vi "Check if Error Occurred.vi"(8 "error in (no error)":errorcluster, 11 "Response header":string) -> (0 "error out":errorcluster, 2 "500 Error":bool, 3 "Error Occurred":bool)   [LabVIEW 2015, in "NI_AWS_Core.lvlib" / "HTTP Request.lvclass"]
doc: "Check the response header to see if there was an error.\nIf an error is found, the AWS_S3_Get_Call_Result.vi may get the details from the response body."
uses:
  HTTP Request.lvclass
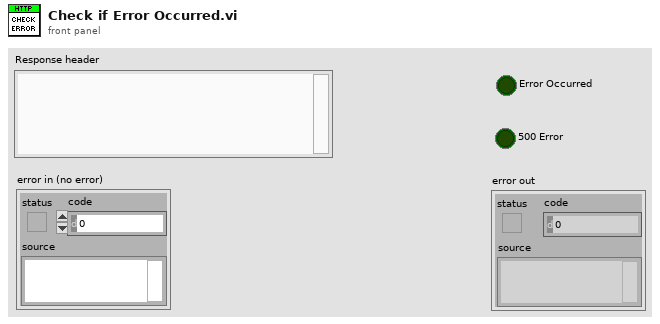
[diagram p1: front panel]
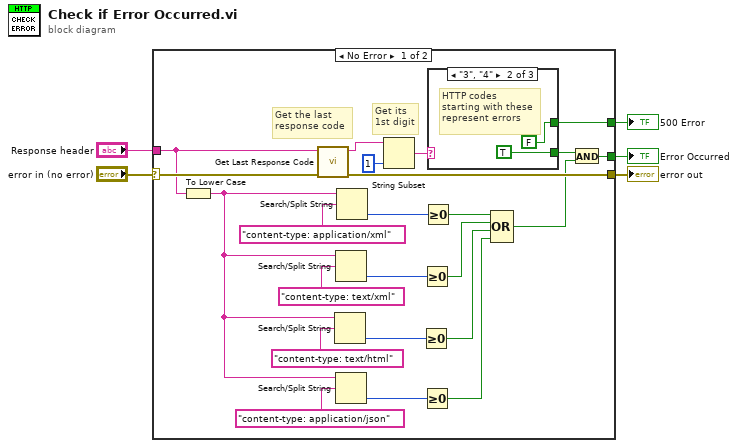
[diagram p0: block diagram]
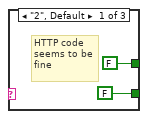
[diagram p2: hidden frame]
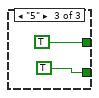
[diagram p3: hidden frame]
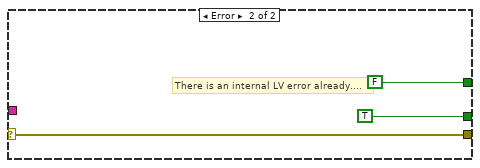
[diagram p4: hidden frame]
diagram:
  n1 = case shown="No Error" "error in (no error)" {
    selector: "error in (no error)" -> [w24 w37]
    tunnel: [w23 w37] -> w3
    tunnel: "Response header" -> [w7 _]
    tunnel: [w25 TRUE] -> w2
    tunnel: [w18 FALSE] -> w1
    frame No Error {
      # "Get its\n1st digit"
      # "Get the last\nresponse code"
      n2 = To Lower Case(string=w7) -> (all lower case string=w6:string)
      n3 = call "Get Last Response Code.vi"("error in (no error)"=w24, "Response header"=w7) -> ("error out"=w23:errorcluster, "Response code (last)"=w22:string)  [unwired: 8 in]
      n4 = Search/Split String(string=w6, search string/char (-)="content-type: text/html") -> (offset of match=w12:i32)  [unwired: 1 in, 2 out]
      n5 = Search/Split String(string=w6, search string/char (-)="content-type: text/xml") -> (offset of match=w17:i32)  [unwired: 1 in, 2 out]
      n6 = Search/Split String(string=w6, search string/char (-)="content-type: application/json") -> (offset of match=w10:i32)  [unwired: 1 in, 2 out]
      n7 = Search/Split String(string=w6, search string/char (-)="content-type: application/xml") -> (offset of match=w27:i32)  [unwired: 1 in, 2 out]
      n8 = String Subset(string=w22, length (rest)=1 ("length (rest)")) -> (substring=w21:string)  [unwired: 1 in]
      n9 = Greater Or Equal To 0?(x=w12) -> (x >= 0?=w11:bool)
      n10 = Greater Or Equal To 0?(x=w17) -> (x >= 0?=w14:bool)
      n11 = Greater Or Equal To 0?(x=w10) -> (x >= 0?=w8:bool)
      n12 = Greater Or Equal To 0?(x=w27) -> (x >= 0?=w19:bool)
      n13 = case shown="\"3\", \"4\"" w21 {
        tunnel: [FALSE TRUE TRUE] -> w26
        tunnel: [FALSE FALSE TRUE] -> w18
        frame "2", Default {
          # "HTTP code\nseems to be\nfine"
        }
        frame "3", "4" {
          # "HTTP codes\nstarting with these\nrepresent errors"
        }
        frame "5" {
        }
      }
      n14 = Compound Arithmetic op=OR(w19, w14, w11, w8) -> (w15:bool)
      n15 = And(x=w26, y=w15) -> (x .and. y?=w25:bool)
    }
    frame Error {
      # "There is an internal LV error already...."
    }
  }
  "Error Occurred" <- w2
  "error out" <- w3
  "500 Error" <- w1
